vi "CSE - Link Source Script Offset to Statement.vi"(8 "error in":errorcluster, 10 "Offset (0)":i32, 11 "CSE RefNum":T1) -> (0 "error out":errorcluster, 1 "Stm Index":i32, 2 "dup Offset":i32=1, 3 "dup CSE RefNum":T1)   [LabVIEW 2021]
doc: "This VI returns the index of the statement in a parsed script that closest matches the specified offset in the source script. If no suitable statement is found, the VI returns -1. Refer to the VI help for more details.\n\n::: CalcExpress Toolkit :::\nCopyright (c) 2000-2026 Konstantin Shifershteyn. All rights reserved."
uses:
  CSE Instance RefNum.ctl
  cersrc/celveng32.dll
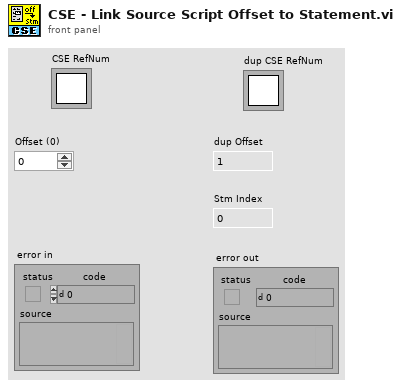
[diagram p1: front panel]
types:
  T1 = typedef "CSE Instance RefNum.ctl" = refnum<k1>
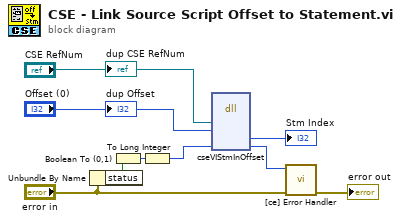
[diagram p0: block diagram]
diagram:
  n1 = Unbundle By Name("error in") -> ("status"=w8:bool)
  n2 = Boolean To (0,1)(Boolean=w8) -> (0, 1=w9:i16)
  n3 = To Long Integer(number=w9) -> (32bit integer=w5:i32)
  n4 = dll-call lib="C:/LV Projects/CalcExpress 40 LV2021/vi.lib/addons/CalcExpress/cersrc/celveng*.dll" fn="cseVIStmInOffset"("iCESP"="CSE RefNum", "Offset"="Offset (0)", "errStat"=w5) -> ("StmIdx"=→"Stm Index":i32, "errStat"=w4:i32)  [unwired: 7 in, 2 out]
  n5 = call "[ce] Error Handler.vi"("error in"="error in", "error code"=w4) -> ("error out"=→"error out":errorcluster)  [unwired: 8 in, 1 out]
  "dup CSE RefNum" <- "CSE RefNum"
  "dup Offset" <- "Offset (0)"
